vi "Create Valve.vi"(5 "Group":refnum<class "Group DBL.lvclass">, 8 "error in (no error)":errorcluster, 10 "Config Element":refnum<class "Config Element.lvclass">, 11 "ValveControlModule in":refnum<class "DigitalControlModule.lvclass">) -> (0 "error out":errorcluster, 3 "ValveControlModule out":refnum<class "DigitalControlModule.lvclass">)   [LabVIEW 2020, in "VolatusControl.lvlib" / "DigitalControlModule.lvclass"]
uses:
  DigitalControlModule.lvclass
  C:/dev/lv20CE/relink/lv-volatus/Volatus/Module/Module.lvclass
  lv-cdm/CDM-Config/Config Element/Config Element.lvclass
  lv-vecto/Vecto/Group DBL/Group DBL.lvclass
  VolatusConfig/Meta Type.ctl
  Volatus/Module/Module.lvclass/Module.ctl
  DigitalControlModule.lvclass/DigitalControlModule.ctl
  lv-cdm/CDM-Config/Config Lookup/Match Meta.vi
  lv-cdm/CDM-Config/Config Element/Owner.vi
  lv-cdm/CDM-Config/Config Manager/Lookup Descendant.vi
  lv-cdm/CDM-Config/Config Filter/Config Lookup.lvclass
  DigitalControl/DigitalControl.lvclass
  Volatus/Module/Module.lvclass
  VolatusConfig/VolatusConfig.lvlib
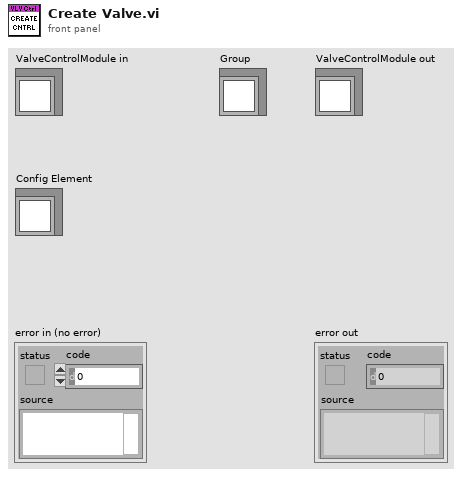
[diagram p1: front panel]
types:
  T1 = typedef "VolatusConfig.lvlib/Meta Type.ctl" = enum16{"UNKNOWN", "VL_System", "VL_Cluster", "VL_Node", "VL_Task", "VL_Group", "VL_Channel", "VL_Task_List", "VL_Scaling", "VL_Sensor", "VL_Sensor_List", "VL_Scale"}
  T2 = map{string, refnum<class "DigitalControl.lvclass">}
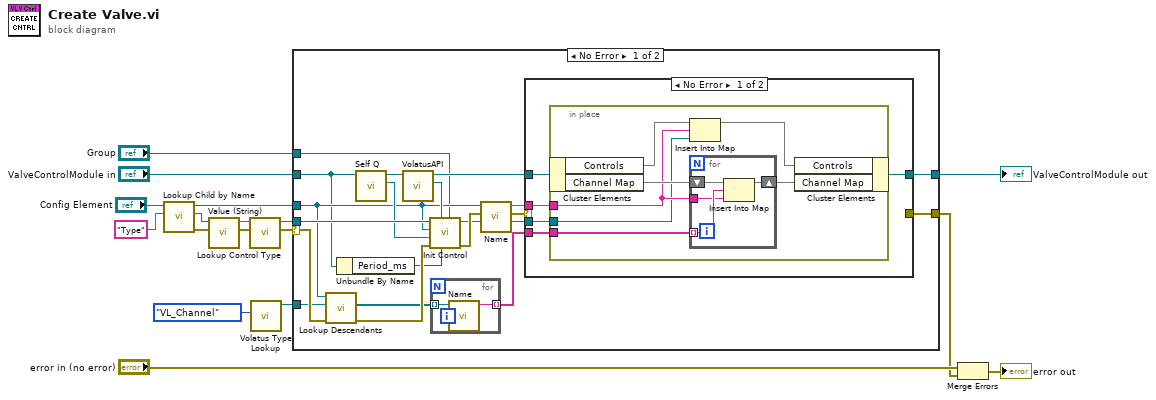
[diagram p0: block diagram]
diagram:
  n1 = call "Lookup Child by Name.vi"("Name"="Type", "Config Element in"="Config Element") -> ("error out"=w12:errorcluster, "Child"=w13:refnum<class "Config Element.lvclass">, "Config Element out"=w7:refnum<class "Config Element.lvclass">)  [unwired: 6 in, 1 out]
  n2 = call "Value (String).vi"("error in (no error)"=w12, "Config Element in"=w13) -> ("error out"=w10:errorcluster, "String Value"=w11:string)  [unwired: 8 in]
  n3 = call "Lookup Control Type.vi"("error in (no error)"=w10, "Control Type"=w11) -> ("error out"=w6:errorcluster, "ValveControl"=w9:refnum<class "DigitalControl.lvclass">)  [unwired: 8 in]
  n4 = call "Volatus Type Lookup.vi"("Meta Type"=Meta_Type."VL_Channel") -> ("Config Lookup out"=w4:refnum<class "Config Lookup.lvclass">)  [unwired: 9 in, 1 out]
  n5 = case shown="No Error" w6 {
    selector: w6 -> [w37 w58]
    tunnel: "ValveControlModule in" -> [w19 w59]
    tunnel: w9 -> [w36 _]
    tunnel: [w23 w59] -> w8
    tunnel: w7 -> [w30 _]
    tunnel: w4 -> [w32 _]
    tunnel: [w21 w58] -> w2
    tunnel: "Group" -> [w20 _]
    frame No Error {
      n6 = call "Lookup Descendants.vi"("error in (no error)"=w37, "Lookup"=w32, "Config Element in"=w30) -> ("error out"=w31:errorcluster, "Descendants"=w28:refnum<class "Config Element.lvclass">[])  [unwired: 6 in, 1 out]
      n7 = Unbundle By Name(w19) -> ("Period_ms"=w18:i64)
      n8 = call "Self Q.vi"("Module in"=w19) -> ("Self Q"=w33:refnum<class "MessageQ.lvclass">, "Module out"=w34:refnum<class "DigitalControlModule.lvclass">)  [unwired: 9 in]
      n9 = call "VolatusAPI.vi"("Module in"=w34) -> ("VolatusAPI"=w35:refnum<class "VolatusAPI.lvclass">, "Module out"=w27:refnum<class "DigitalControlModule.lvclass">)  [unwired: 9 in]
      n10 = call-dynamic "Init Control.vi"("Group"=w20, "Period ms"=w18, "VolatusAPI"=w35, "error in (no error)"=w31, "Control MsgQ"=w33, "Config Element"=w30, "Valve in"=w36) -> ("error out"=w29:errorcluster, "Valve out"=w24:refnum<class "DigitalControl.lvclass">)  [unwired: 3 in]
      n11 = for {
        tunnel: w28 -> [w57] mode=indexing
        tunnel: [w56] -> w25 mode=indexing
        n12 = call "Name.vi"("Config Element in"=w57) -> ("Name"=w56:string)  [unwired: 9 in, 1 out]
      }
      n13 = call "Name.vi"("error in (no error)"=w29, "Config Element in"=w30) -> ("error out"=w22:errorcluster, "Name"=w26:string)  [unwired: 8 in]
      n14 = case shown="No Error" w22 {
        selector: w22 -> [_ w55]
        tunnel: w27 -> [w42 w54]
        tunnel: w26 -> [w41 _]
        tunnel: w25 -> [w40 _]
        tunnel: w24 -> [w39 _]
        tunnel: [w38 w54] -> w23
        tunnel: [_ w55] -> w21
        frame No Error {
          n15 = in-place {
            in-place-border: w41 -> [w46]
            in-place-border: w40 -> [w45]
            in-place-border: w39 -> [w43]
            n16 = in-place-cluster #1(w42) -> ("Controls"=w49:T2, "Channel Map"=w47:map{string, string})
            n17 = Insert Into Map(map in=w49, key=w46, value=w43) -> (map out=w48:T2)  [unwired: 2 out]
            n18 = for {
              shift-right: [w50] -> w44
              shift-left: w47 -> [w53]
              tunnel: w46 -> [w51]
              tunnel: w45 -> [w52] mode=indexing
              n19 = Insert Into Map(map in=w53, key=w52, value=w51) -> (map out=w50:map{string, string})  [unwired: 2 out]
            }
            n20 = in-place-cluster #1("Controls"=w48, "Channel Map"=w44) -> (w38:refnum<class "DigitalControlModule.lvclass">)
          }
        }
        frame Error {
        }
      }
    }
    frame Error {
    }
  }
  "ValveControlModule out" <- w8
  n21 = Merge Errors("error in (no error)", w2) -> (→"error out":errorcluster)
